vi "WLAN_SigContent2.vi"(8 "error in (no error)":errorcluster, 10 "Frequency channel estimation":cdb[](array[numeric]) format="%.6g", 11 "SIG":cdb[](array[numeric])) -> (0 "error out":errorcluster, 3 "Alpha":u32, 4 "Modulation parameter LP":T1, 5 "SIG valid?":bool)   [LabVIEW 2022 SP3]
panel:
  out "size(s) 2":i32
  out "size(s)":i32
  out "output bit stream":i8[](array[numeric])
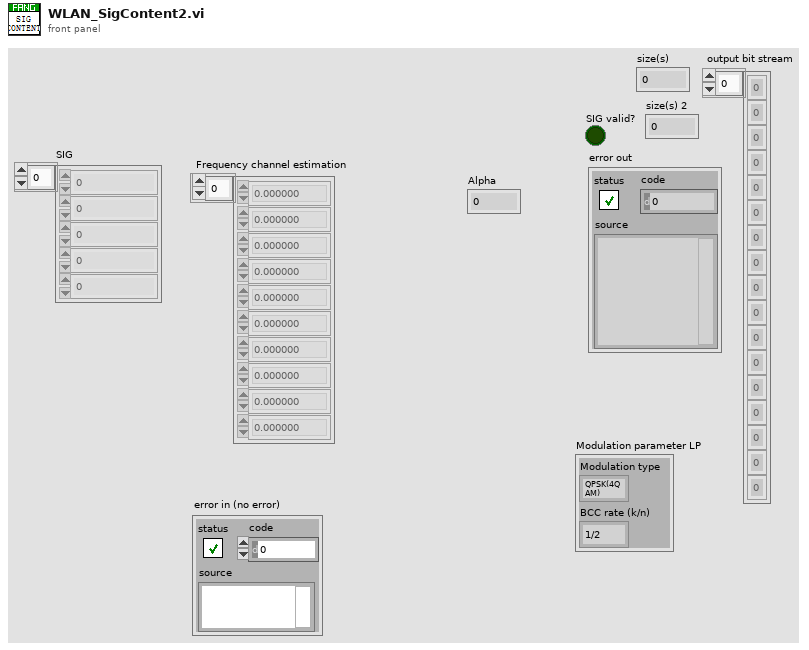
[diagram p1: front panel]
types:
  T1 = cluster{"Modulation type":enum16{"QPSK(4QAM)", "64QAM", "16QAM", "BPSK"}, "BCC rate (k/n)":enum16{"1/2", "2/3", "3/4"}}
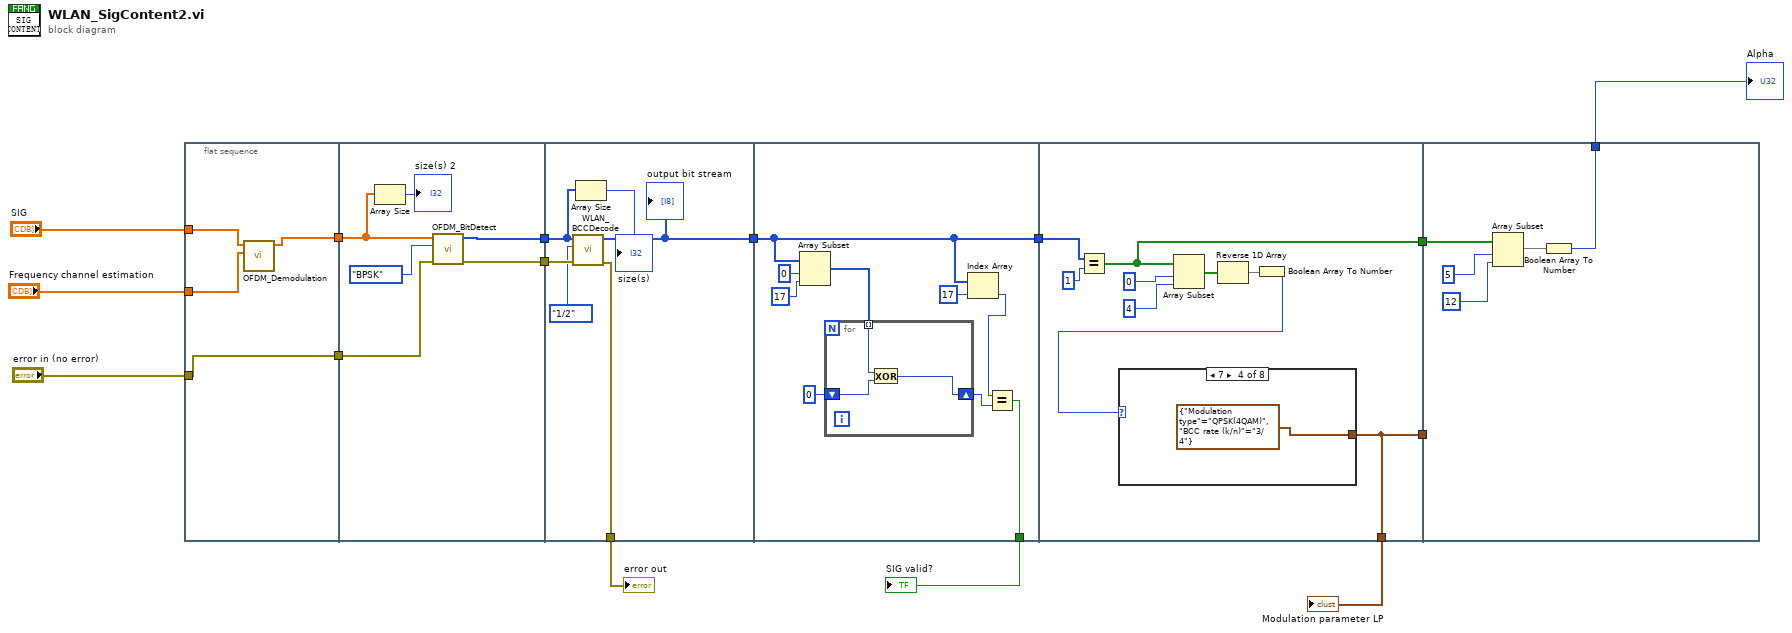
[diagram p0: block diagram]
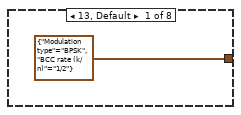
[diagram p2: hidden frame]
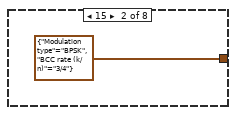
[diagram p3: hidden frame]
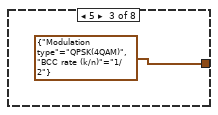
[diagram p4: hidden frame]
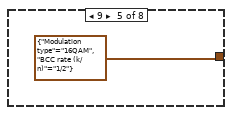
[diagram p5: hidden frame]
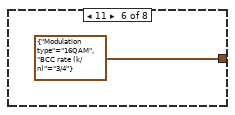
[diagram p6: hidden frame]
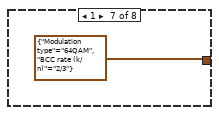
[diagram p7: hidden frame]
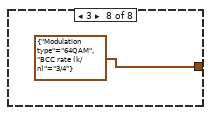
[diagram p8: hidden frame]
diagram:
  n1 = flat-sequence {
    tunnel: [w19] -> w15
    tunnel: "SIG" -> [w18]
    tunnel: "Frequency channel estimation" -> [w17]
    tunnel: [w16] -> w9
    tunnel: "error in (no error)" -> [w16]
    tunnel: w15 -> [w22]
    tunnel: [w25] -> w12
    tunnel: [w24] -> w10
    tunnel: w9 -> [w23]
    tunnel: w12 -> [w28]
    tunnel: [w31] -> w6
    tunnel: w10 -> [w30]
    tunnel: [w29] -> w2
    tunnel: w6 -> [w37]
    tunnel: [w37] -> w5
    tunnel: [w33] -> w1
    tunnel: w5 -> [w51]
    tunnel: [w48] -> w11
    tunnel: [w44] -> w4
    tunnel: [w44] -> w3
    tunnel: w11 -> [w63]
    tunnel: [w61] -> w7
    tunnel: w3 -> [_]
    frame #0 {
      n2 = call "OFDM_Demodulation.vi"("Frequency channel estimation"=w17, "Input sequence"=w18) -> ("Output sequence"=w19:cdb[])  [unwired: 9 in]
    }
    frame #1 {
      n3 = Array Size(array=w22) -> (size(s)=→"size(s) 2":i32)
      n4 = call "OFDM_BitDetect.vi"("Input symbols"=w22, "Modulation type"=enum16{"QPSK(4QAM)", "64QAM", "16QAM", "BPSK"}."BPSK", "error in (no error)"=w23) -> ("Output bits"=w25:i8[], "error out"=w24:errorcluster)  [unwired: 6 in]
    }
    frame #2 {
      n5 = call "WLAN_BCCDecode.vi"("error in (no error)"=w30, "BCC rate (k/n)"=enum16{"1/2", "2/3", "3/4"}."1/2", "input bit stream"=w28) -> ("error out"=w29:errorcluster, "output bit stream"=w31:i8[])  [unwired: 7 in]
      "output bit stream" <- w31
      n6 = Array Size(array=w28) -> (size(s)=→"size(s)":i32)
    }
    frame #3 {
      n7 = Array Subset(array=w37, index=0, length=17) -> (w39:i8[])
      n8 = for {
        shift-right: [w42] -> w34
        shift-left: i8 0 -> [w43]
        tunnel: w39 -> [w41] mode=indexing
        n9 = Exclusive Or(1:w43, 2:w41) -> (0:w42:i8)
      }
      n10 = Index Array(array=w37, index=17) -> (element=w35:i8)
      n11 = Equal?(x=w35, y=w34) -> (x = y?=w33:bool)
    }
    frame #4 {
      n12 = Equal?(x=w51, y=1 ("length")) -> (x = y?=w48:bool[])
      n13 = Array Subset(array=w48, index=0, length=4) -> (w47:bool[])
      n14 = Reverse 1D Array(array=w47) -> (reversed array=w46:bool[])
      n15 = Boolean Array To Number(Boolean array=w46) -> (number=w45:u32)
      n16 = case shown="7" w45 {
        tunnel: [T1 {"Modulation type"=enum."BPSK", "BCC rate (k/n)"=enum."1/2"} ("Modulation parameter") T1 {"Modulation type"=enum."BPSK", "BCC rate (k/n)"=enum."3/4"} ("Modulation parameter") T1 {"Modulation type"=enum."QPSK(4QAM)", "BCC rate (k/n)"=enum."1/2"} ("Modulation parameter") T1 {"Modulation type"=enum."QPSK(4QAM)", "BCC rate (k/n)"=enum."3/4"} ("Modulation parameter") T1 {"Modulation type"=enum."16QAM", "BCC rate (k/n)"=enum."1/2"} ("Modulation parameter") T1 {"Modulation type"=enum."16QAM", "BCC rate (k/n)"=enum."3/4"} ("Modulation parameter") T1 {"Modulation type"=enum."64QAM", "BCC rate (k/n)"=enum."2/3"} ("Modulation parameter") T1 {"Modulation type"=enum."64QAM", "BCC rate (k/n)"=enum."3/4"} ("Modulation parameter")] -> w44
        frame 13, Default {
        }
        frame 15 {
        }
        frame 5 {
        }
        frame 7 {
        }
        frame 9 {
        }
        frame 11 {
        }
        frame 1 {
        }
        frame 3 {
        }
      }
    }
    frame #5 {
      n17 = Array Subset(array=w63, index=5, length=12) -> (w62:bool[])
      n18 = Boolean Array To Number(Boolean array=w62) -> (number=w61:u32)
    }
  }
  "Alpha" <- w7
  "Modulation parameter LP" <- w4
  "error out" <- w2
  "SIG valid?" <- w1
